vi "Get SMS Attributes.vi"(8 "error in (no error)":errorcluster, 11 "SMS in":refnum<class "SMS.lvclass">) -> (0 "error out":errorcluster, 2 "SMS Attributes":T1[](array[typedef]), 3 "SMS out":refnum<class "SMS.lvclass">)   [LabVIEW 2015, in "NI_AWS_SNS.lvlib" / "SMS.lvclass"]
doc: "Returns the settings for sending SMS messages from your account.\n\nThese settings are set with the Set SMS Attributes action."
uses:
  SMS.lvclass
  SMS Attribute Value Pair.ctl
  SMS Attribute.ctl
  Core/HTTP Request/Request Options.ctl
  Core/HTTP Request/Name Value Pair.ctl
  Core/HTTP Request/Region handling.ctl
  Core/HTTP Request/URL formatting.ctl
  Core/HTTP Request/HTTP Request.lvclass
  XML Parsing/NI_XML Parsing.lvlib
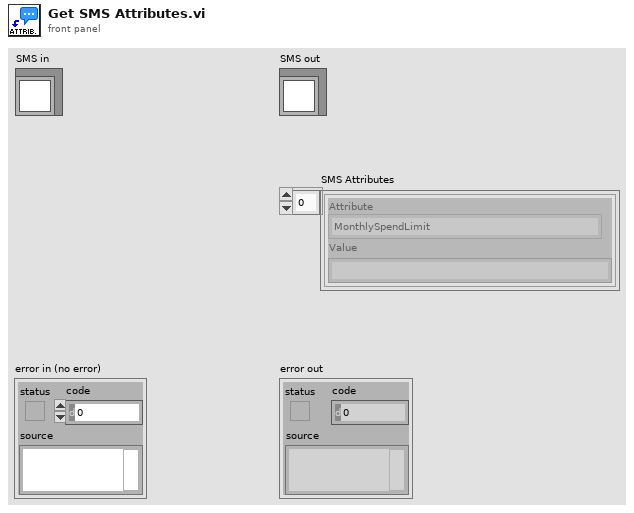
[diagram p1: front panel]
types:
  T1 = typedef "NI_AWS_SNS.lvlib/SMS.lvclass/SMS Attribute Value Pair.ctl" = cluster{"Attribute":T2, "Value":string}
  T2 = typedef "NI_AWS_SNS.lvlib/SMS.lvclass/SMS Attribute.ctl" = enum16{"MonthlySpendLimit", "DeliveryStatusIAMRole", "DeliveryStatusSuccessSamplingRate", "DefaultSenderID", "DefaultSMSType", "UsageReportS3Bucket"}
  T3 = typedef "NI_AWS_Core.lvlib/HTTP Request.lvclass/Name Value Pair.ctl" = cluster{"name":string, "value":string}
  T4 = typedef "NI_AWS_Core.lvlib/HTTP Request.lvclass/Request Options.ctl" = cluster{"request headers":T3[], "request parameters":T3[], "request body":string, "region handling":T5, "URL formatting":T6}
  T5 = typedef "NI_AWS_Core.lvlib/HTTP Request.lvclass/Region handling.ctl" = enum16{"use region everywhere", "use region (authentication only)", "use region (URL only)", "ignore region everwhere"}
  T6 = typedef "NI_AWS_Core.lvlib/HTTP Request.lvclass/URL formatting.ctl" = enum16{"region-", "region."}
  T7 = typedef "NI_AWS_Core.lvlib/HTTP Request.lvclass/Response.ctl" = cluster{"Headers":string, "Body":string}
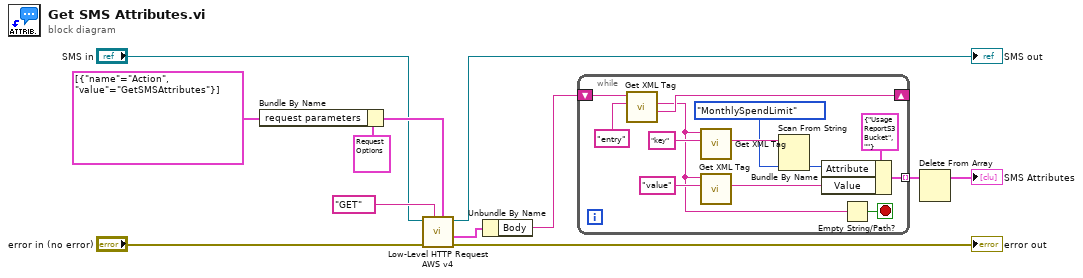
[diagram p0: block diagram]
diagram:
  n1 = Bundle By Name(cluster=T4 {"request headers"=[], "request parameters"=[], "request body"="", "region handling"=enum."use region everywhere", "URL formatting"=enum."region."} ("Request Options"), "request parameters"=T3[] [{"name"="Action", "value"="GetSMSAttributes"}]) -> (w4:T4)
  n2 = call "Low-Level HTTP Request AWS v4.vi"("Request Options"=w4, "HTTP-Verb"="GET", "error in (no error)"="error in (no error)", "AWS Core in"="SMS in") -> ("error out"=→"error out":errorcluster, "Response"=w5:T7, "AWS Core out"=→"SMS out":refnum<class "SMS.lvclass">)  [unwired: 4 in, 1 out]
  n3 = Unbundle By Name(w5) -> ("Body"=w8:string)
  n4 = while {
    shift-right: [w24] -> _
    shift-left: w8 -> [w25]
    tunnel: [w19] -> w7 mode=indexing
    stop <- w17 stop-if-true
    n5 = call "Get XML Tag.vi"("Tag name"="entry", "XML String in"=w25) -> ("Remaining string"=w24:string, "Tag value"=w18:string)  [unwired: 5 in, 3 out]
    n6 = call "Get XML Tag.vi"("Tag name"="key", "XML String in"=w18) -> ("Tag value"=w15:string)  [unwired: 5 in, 4 out]
    n7 = call "Get XML Tag.vi"("Tag name"="value", "XML String in"=w18) -> ("Tag value"=w20:string)  [unwired: 5 in, 4 out]
    n8 = Scan From String(input string=w15, default 1=SMS_Attribute."MonthlySpendLimit" ("Attribute")) -> (output 1=w13:T2)  [unwired: 3 in, 3 out]
    n9 = Bundle By Name(cluster=T1 {"Attribute"=enum."UsageReportS3Bucket", "Value"=""} ("SMS Attribute Value Pair"), "Attribute"=w13, "Value"=w20) -> (w19:T1)
    n10 = Empty String/Path?(string/path=w18) -> (empty?=w17:bool)
  }
  n11 = Delete From Array(array=w7) -> (array with subset deleted=→"SMS Attributes":T1[])  [unwired: 2 in, 1 out]
